vi "Table Buffer - Dequeue.vi"(8 "error in (no error)":errorcluster) -> (0 "error out":errorcluster, 3 "Data":string[][](array[string]))   [LabVIEW 2025, in "I2C Bus Monitor UI.lvlib"]
uses:
  I2C Bus Monitor UI.lvlib
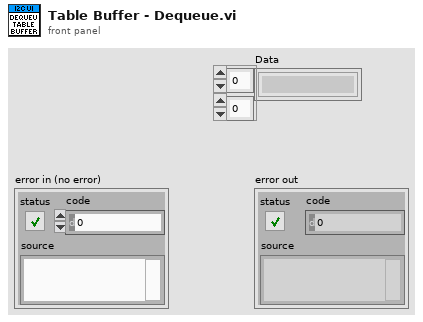
[diagram p1: front panel]
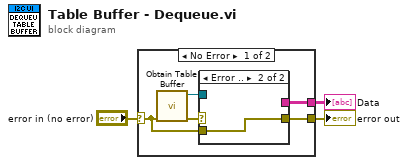
[diagram p0: block diagram]
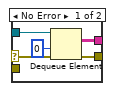
[diagram p2: hidden frame]
diagram:
  n1 = case shown="No Error" "error in (no error)" {
    selector: "error in (no error)" -> [w4 w15]
    tunnel: [w8 w15] -> w2
    tunnel: [w7 _] -> w1
    frame No Error {
      n2 = call "Obtain Table Buffer.vi"("error in (no error)"=w4) -> ("error out"=w6:errorcluster, "Table Queue"=w5:refnum<queue>)  [unwired: 9 in]
      n3 = case shown="Error .." w6 {
        selector: w6 -> [w10 _]
        tunnel: [w13 w14] -> w8
        tunnel: [w12 _] -> w7
        tunnel: w5 -> [w9 _]
        tunnel: w4 -> [_ w14]
        frame No Error {
          n4 = Dequeue Element(queue=w9, timeout in ms (-1)=0, error in (no error)=w10) -> (element=w12:string[][], error out=w13:errorcluster)  [unwired: 2 out]
        }
        frame Error {
        }
      }
    }
    frame Error {
    }
  }
  "error out" <- w2
  "Data" <- w1
